vi "query NR UL_DL Channel Bandwidth.vi"(8 "error in (no error)":errorcluster, 9 "Direction":T1, 10 "Bandwidth Setting Param":T2, 11 "Anritsu Call Box_Implement in":refnum<class "Anritsu Call Box_Implement.lvclass">) -> (0 "error out":errorcluster, 2 "BW (MHz)":u32, 3 "Anritsu Call Box_Implement out":refnum<class "Anritsu Call Box_Implement.lvclass">)   [LabVIEW 2023, in "ANRITSU Call Box.lvlib" / "Anritsu Call Box_Implement.lvclass"]
uses:
  Anritsu Call Box_Implement.lvclass
  Anritsu Call Box_Implement.lvclass/Anritsu Call Box_Implement.ctl
  NR/NR.lvclass
  Type Definition/NR Channel Bandwidth Param.ctl
  ANRITSU Call Box.lvlib
  Type Definition/Uplink Downlink Enum.ctl
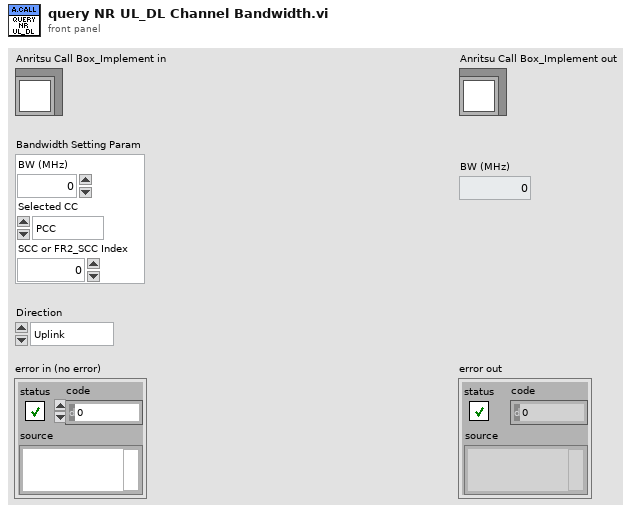
[diagram p1: front panel]
types:
  T1 = typedef "ANRITSU Call Box.lvlib/Uplink Downlink Enum.ctl" = enum16{"Uplink", "Downlink"}
  T2 = typedef "ANRITSU Call Box.lvlib/NR Channel Bandwidth Param.ctl" = cluster{"BW (MHz)":u32, "Selected CC":enum16{"PCC", "SCC", "FR2_PCC", "FR2_SCC"}, "SCC or FR2_SCC Index":u32}
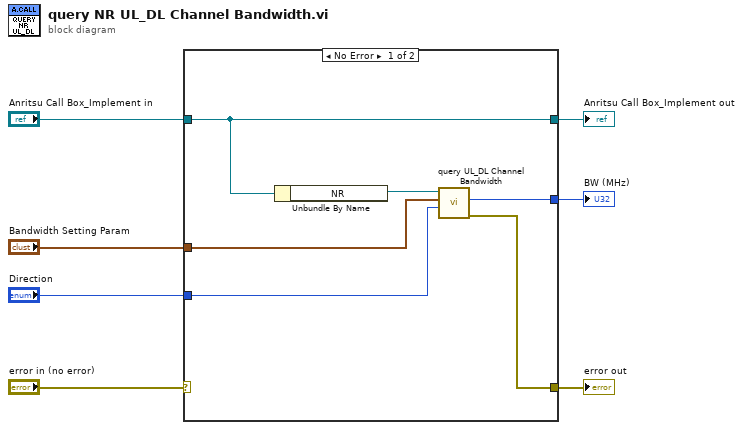
[diagram p0: block diagram]
diagram:
  n1 = case shown="No Error" "error in (no error)" {
    selector: "error in (no error)" -> [_ w14]
    tunnel: "Anritsu Call Box_Implement in" -> [w13 w15]
    tunnel: [w13 w15] -> w7
    tunnel: [w9 w14] -> w4
    tunnel: "Direction" -> [w10 _]
    tunnel: "Bandwidth Setting Param" -> [w11 _]
    tunnel: [w8 _] -> w1
    frame No Error {
      n2 = Unbundle By Name(w13) -> ("NR"=w12:refnum<class "NR.lvclass">)
      n3 = call "query UL_DL Channel Bandwidth.vi"("Direction"=w10, "Bandwidth Setting Param"=w11, "NR in"=w12) -> ("error out"=w9:errorcluster, "BW (MHz)"=w8:u32)  [unwired: 6 in, 1 out]
    }
    frame Error {
    }
  }
  "error out" <- w4
  "Anritsu Call Box_Implement out" <- w7
  "BW (MHz)" <- w1
